vi "ConfigSSL Verify False.vi"(11 "error in":errorcluster) -> (15 "error out":errorcluster)   [LabVIEW 2024]
doc: "Static analysis fixture with verify server false and a permanent false guard."
uses:
  <vilib>/httpClient/LabVIEWHTTPClient.lvlib
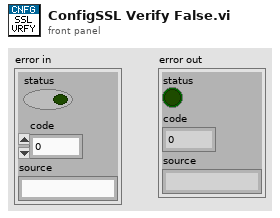
[diagram p1: front panel]
types:
  T1 = typedef "LabVIEWHTTPClient.lvlib/ClientHandle.ctl" = refnum<k1>
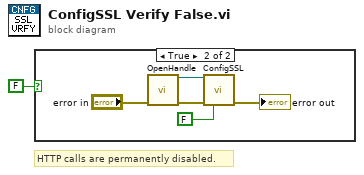
[diagram p0: block diagram]
diagram:
  # "HTTP calls are permanently disabled."
  n1 = case shown="True" FALSE ("guard") {
    frame False {
    }
    frame True {
      n2 = call <vilib>:"OpenHandle.vi"("error in (no error)"="error in") -> ("client handle out"=w3:T1, "error out"=w4:errorcluster)  [unwired: 13 in]
      n3 = call <vilib>:"ConfigSSL.vi"("client handle"=w3, "error in (no error)"=w4, "verify server (true)"=FALSE ("verify server")) -> ("error out"=→"error out":errorcluster)  [unwired: 11 in, 1 out]
    }
  }
